vi "FTCU Adjust.vi"(8 "error in":errorcluster, 11 "DAC FTCU in":refnum<class "DAC FTCU.lvclass">) -> (0 "error out":errorcluster, 3 "DAC FTCU out":refnum<class "DAC FTCU.lvclass">)   [LabVIEW 2019, in "DAC.lvlib" / "DAC FTCU.lvclass"]
uses:
  DAC FTCU.lvclass
  DAC FTCU.lvclass/DAC FTCU.ctl
  Results/DeepU Results/DeepU Results.lvclass/DeepU Results.ctl
  Results/Results Method.ctl
  Results/Results.lvlib
  Results/DeepU Results/DeepU Results.lvclass
  DAC.lvclass
  C:/Users/wg/Documents/LV_Projects/test-stand/App/DAC/DAC.lvclass
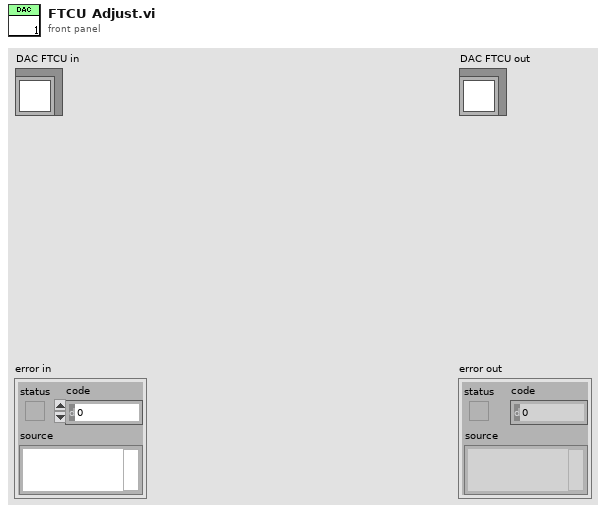
[diagram p1: front panel]
types:
  T1 = typedef "Results.lvlib/Results Method.ctl" = enum16{"Get", "Set"}
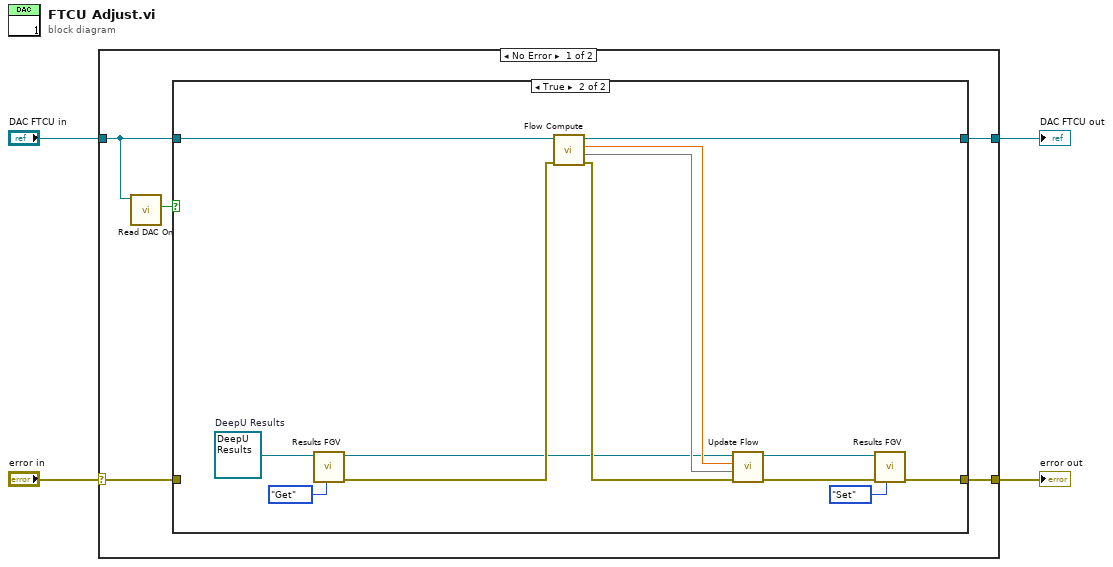
[diagram p0: block diagram]
diagram:
  n1 = case shown="No Error" "error in" {
    selector: "error in" -> [w6 w26]
    tunnel: [w5 w26] -> w3
    tunnel: [w7 w25] -> w1
    tunnel: "DAC FTCU in" -> [w8 w25]
    frame No Error {
      n2 = call "Read DAC On.vi"("DAC in"=w8) -> ("DAC On"=w9:bool)  [unwired: 8 in, 2 out]
      n3 = case shown="True" w9 {
        tunnel: w8 -> [w11 w20]
        tunnel: [w11 w19] -> w7
        tunnel: w6 -> [w10 _]
        tunnel: [w10 w21] -> w5
        frame False {
        }
        frame True {
          w24 = refnum<class "DeepU Results.lvclass"> refnum  # DeepU Results
          n4 = call-dynamic "Results FGV.vi"("Method"=Results_Method."Get", "DeepU Results in"=w24) -> ("error out"=w16:errorcluster, "DeepU Results out"=w13:refnum<class "DeepU Results.lvclass">)  [unwired: 8 in]
          n5 = call "Flow Compute.vi"("error in"=w16, "DAC FTCU in"=w20) -> ("error out"=w15:errorcluster, "Status"=w18:map{string, bool}, "Flow"=w17:sgl, "DAC FTCU out"=w19:refnum<class "DAC FTCU.lvclass">)  [unwired: 6 in]
          n6 = call "Update Flow.vi"("error in"=w15, "Status"=w18, "Flow"=w17, "DeepU Results in"=w13) -> ("error out"=w14:errorcluster, "DeepU Results out"=w12:refnum<class "DeepU Results.lvclass">)  [unwired: 6 in]
          n7 = call-dynamic "Results FGV.vi"("Method"=Results_Method."Set", "error in"=w14, "DeepU Results in"=w12) -> ("error out"=w21:errorcluster)  [unwired: 7 in, 1 out]
        }
      }
    }
    frame Error {
    }
  }
  "error out" <- w3
  "DAC FTCU out" <- w1
